vi "App Start.vi"(8 "error in (no error)":errorcluster, 10 "Core APIs":T1, 11 "DemoApp in":refnum<class "DemoApp.lvclass">) -> (0 "error out":errorcluster, 3 "DemoApp out":refnum<class "DemoApp.lvclass">)   [LabVIEW 2020, in "VolatusDemo.lvlib" / "DemoApp.lvclass"]
uses:
  DemoApp.lvclass
  VolatusData/LoggingAPI/LoggingAPI.lvclass
  Volatus/VolatusAPI/VolatusAPI.lvclass
  C:/dev/lv20CE/relink/lv-volatus/Volatus/LoggingAPI/LoggingAPI.lvclass
  C:/dev/lv20CE/relink/lv-volatus/Volatus/API/API.lvclass
  Volatus/Core APIs.ctl
  Volatus/Volatus.lvlib
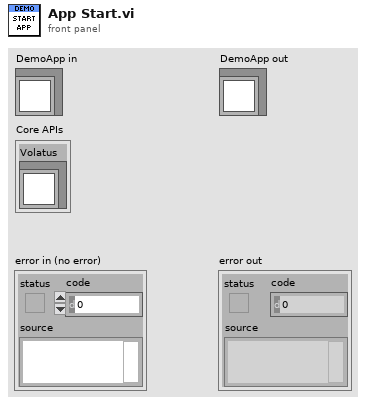
[diagram p1: front panel]
types:
  T1 = typedef "Volatus.lvlib/Core APIs.ctl" = cluster{"Volatus":refnum<class "VolatusAPI.lvclass">}
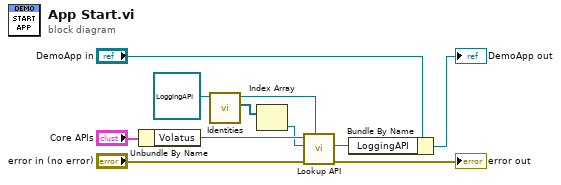
[diagram p0: block diagram]
diagram:
  n1 = Unbundle By Name("Core APIs") -> ("Volatus"=w9:refnum<class "VolatusAPI.lvclass">)
  n2 = call-dynamic "Identities.vi"("LoggingAPI in"=refnum<class "LoggingAPI.lvclass"> refnum ("VolatusDataLogger:LoggingAPI.lvclass")) -> ("Identities"=w6:refnum<class "Identity.lvclass">[], "LoggingAPI out"=w7:refnum<class "LoggingAPI.lvclass">)  [unwired: 8 in, 1 out]
  n3 = Index Array(array=w6) -> (element=w5:refnum<class "Identity.lvclass">)  [unwired: 1 in]
  n4 = call "Lookup API.vi"("API Type"=w7, "error in (no error)"="error in (no error)", "Identity"=w5, "VolatusAPI in"=w9) -> ("error out"=→"error out":errorcluster, "API Type"=w1:refnum<class "LoggingAPI.lvclass">)  [unwired: 5 in, 1 out]
  n5 = Bundle By Name(cluster="DemoApp in", "LoggingAPI"=w1) -> (→"DemoApp out":refnum<class "DemoApp.lvclass">)
